vi "BuildWindTurbineFrame.vi"(2 "LED Flow Speed":dbl min=0.0 max=80.0 step=1.0, 3 "PWM Command":dbl min=0.0 max=255.0 step=1.0, 4 "Wind Speed":dbl min=0.0 max=30.0 step=0.5, 5 "Node Enable":bool) -> (0 "Frame Preview":string, 1 "Frame Bytes":u8[](array[numeric]))   [LabVIEW 2025]
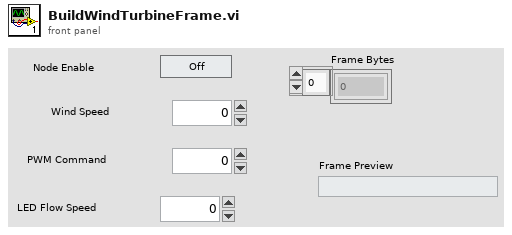
[diagram p1: front panel]
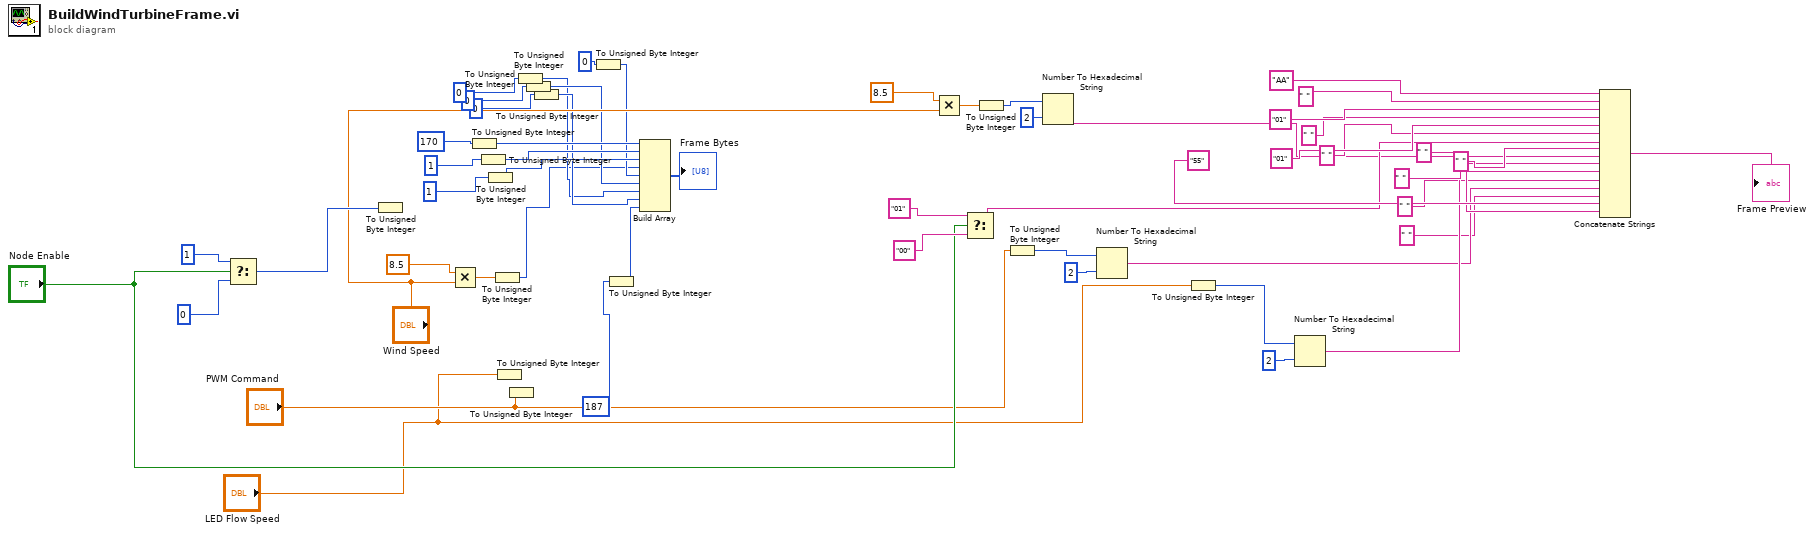
[diagram p0: block diagram]
diagram:
  n1 = Select(t=1, s="Node Enable", f=0) -> (s? t:f=w43:i32)
  n2 = To Unsigned Byte Integer(number=w43) -> ()  [unwired: 1 out]
  n3 = Multiply(x=8.5, y="Wind Speed") -> (x*y=w49:dbl)
  n4 = To Unsigned Byte Integer(number=170) -> (unsigned 8bit integer=w48:u8)
  n5 = To Unsigned Byte Integer(number=1) -> (unsigned 8bit integer=w47:u8)
  n6 = To Unsigned Byte Integer(number=1) -> (unsigned 8bit integer=w46:u8)
  n7 = To Unsigned Byte Integer(number=w49) -> (unsigned 8bit integer=w1:u8)
  n8 = To Unsigned Byte Integer(number="LED Flow Speed") -> ()  [unwired: 1 out]
  n9 = To Unsigned Byte Integer(number="PWM Command") -> ()  [unwired: 1 out]
  n10 = To Unsigned Byte Integer(number=0) -> (unsigned 8bit integer=w3:u8)
  n11 = To Unsigned Byte Integer(number=0) -> (unsigned 8bit integer=w4:u8)
  n12 = To Unsigned Byte Integer(number=0) -> (unsigned 8bit integer=w5:u8)
  n13 = To Unsigned Byte Integer(number=0) -> (unsigned 8bit integer=w6:u8)
  n14 = To Unsigned Byte Integer(number=187) -> (unsigned 8bit integer=w2:u8)
  n15 = Build Array(w48, w47, w46, w1, w6, w4, w3, w5, w2) -> (→"Frame Bytes":u8[])
  n16 = Multiply(x=8.5, y="Wind Speed") -> (x*y=w39:dbl)
  n17 = Select(t="01", s="Node Enable", f="00") -> (s? t:f=w24:string)
  n18 = To Unsigned Byte Integer(number=w39) -> (unsigned 8bit integer=w38:u8)
  n19 = To Unsigned Byte Integer(number="PWM Command") -> (unsigned 8bit integer=w33:u8)
  n20 = Number To Hexadecimal String(1:i16 2 ("width (-)"), 2:w38) -> (0:w22:string)
  n21 = Number To Hexadecimal String(1:i16 2 ("width (-)"), 2:w33) -> (0:w18:string)
  n22 = To Unsigned Byte Integer(number="LED Flow Speed") -> (unsigned 8bit integer=w35:u8)
  n23 = Number To Hexadecimal String(1:i16 2 ("width (-)"), 2:w35) -> (0:w20:string)
  n24 = Concatenate Strings("AA", " ", "01", " ", "01", " ", "55", " ", w24, " ", w22, " ", w20, " ", w18, " ") -> (→"Frame Preview":string)
